vi "Native_GetControlVIType.vi"() -> ()   [LabVIEW 2024]
panel:
  out "error out":errorcluster caption="错误输出"
  out "control_vi_type":T1(ring)
  in  "target_path":path
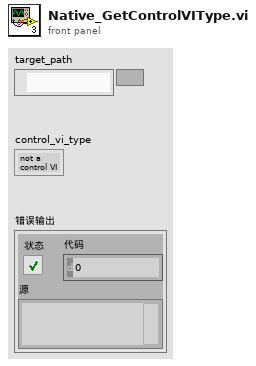
[diagram p1: front panel]
types:
  T1 = enum32{"not a control VI", "control", "typedef", "strict typedef"}
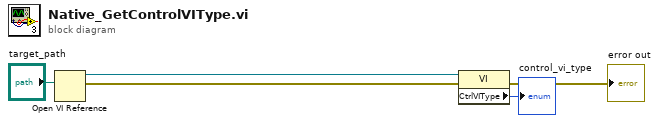
[diagram p0: block diagram]
diagram:
  n1 = Open VI Reference ("打开VI引用")(vi path="target_path") -> (vi reference=w4:refnum<vi>, error out=w3:errorcluster)  [unwired: 5 in]
  n2 = property on="属性节点" class="VI"(reference=w4, error in=w3) -> (error out=→"error out":errorcluster, "CtrlVIType"=→"control_vi_type":T1)  [unwired: 1 out]
